vi "Semaphore Open.vi"(7 "permissions (0664)":T2={"owner"={"read"=TRUE, "write"=TRUE, "execute"=FALSE}, "group"={"read"=TRUE, "write"=TRUE, "execute"=FALSE}, "everyone"={"read"=TRUE, "write"=FALSE, "execute"=FALSE}}, 8 "error in (no error)":errorcluster, 9 "initial value (0)":u32, 10 "file mode (open)":T1, 11 "name":string) -> (0 "error out":errorcluster, 3 "Semaphore out":T3)   [LabVIEW 2016, in "Linux RT IPC.POSIX Threads.lvlib" / "Semaphore.lvclass"]
doc: "Calls sem_open() to open a reference to a named semaphore and returns a pointer.\n\nThis VI initializes the semaphore object and sets its default values.\n\nRefer to online POSIX documentation for more information."
uses:
  Semaphore.lvclass
  Controls/reference.ctl
  Shared Memory/Controls/file mode.ctl
  C/Controls/file creation flags.ctl
  POSIX Thread Object/Private VIs/libpthread path.vi
  C/SubVIs/permission group to mode_t.vi
  C/SubVIs/OR flags U32.vi
  POSIX Thread Object/Private VIs/get pthread error.vi
  <vilib>/NI/NI Linux RT Errno/VIs/Public/SubVIs/errno enum to number.vi
  <vilib>/NI/NI Linux RT Errno/VIs/Public/Get Errno Value for Calling Thread.vi
  POSIX Thread Object/POSIX Thread Object.lvclass
  C/Linux RT IPC.C.lvlib
  Shared Memory/Linux RT IPC.Shared Memory.lvlib
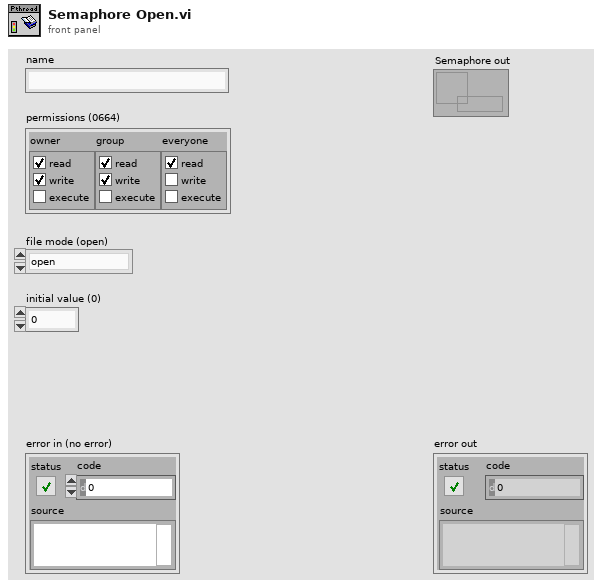
[diagram p1: front panel]
types:
  T1 = typedef "Linux RT IPC.Shared Memory.lvlib/file mode.ctl" = enum16{"open", "create/replace"}
  T2 = cluster{"owner":cluster{"read":bool, "write":bool, "execute":bool}, "group":cluster{"read":bool, "write":bool, "execute":bool}, "everyone":cluster{"read":bool, "write":bool, "execute":bool}}
  T3 = typedef "Linux RT IPC.POSIX Threads.lvlib/Semaphore.lvclass/reference.ctl" = refnum<data-value>
  T4 = typedef "Linux RT IPC.C.lvlib/file creation flags.ctl" = u32
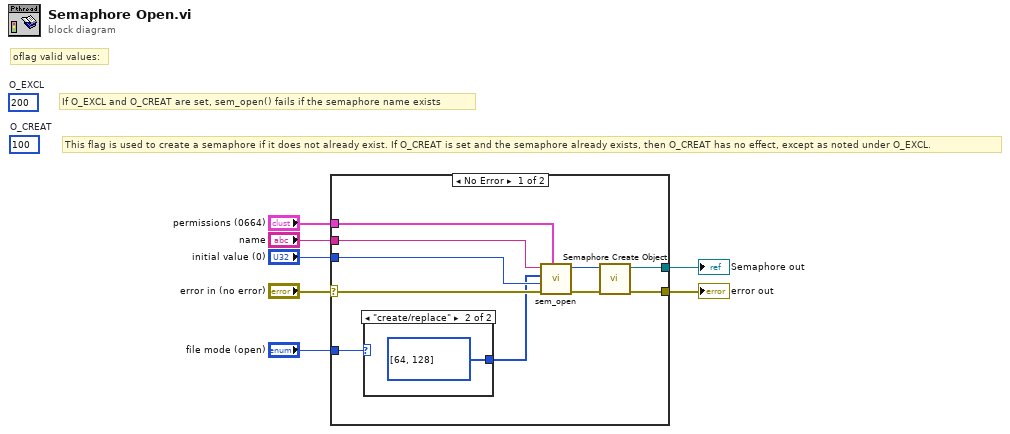
[diagram p0: block diagram]
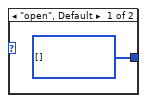
[diagram p2: hidden frame]
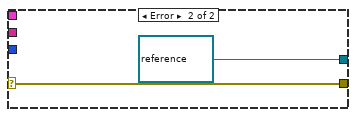
[diagram p3: hidden frame]
diagram:
  (unwired) u32 200  # O_EXCL
  (unwired) u32 100  # O_CREAT
  # "If O_EXCL and O_CREAT are set, sem_open() fails if the semaphore name exists"
  # "This flag is used to create a semaphore if it does not already exist. If O_CREAT is set and the semaphore already exists, then O_CREAT has no effect, except as noted under O_EXCL."
  # "oflag valid values:"
  n1 = case shown="No Error" "error in (no error)" {
    selector: "error in (no error)" -> [w15 w21]
    tunnel: [w11 w21] -> w6
    tunnel: "name" -> [w17 _]
    tunnel: "initial value (0)" -> [w16 _]
    tunnel: "permissions (0664)" -> [w14 _]
    tunnel: [w10 T3 refnum ("Semaphore out")] -> w2
    tunnel: "file mode (open)" -> [w9 _]
    frame No Error {
      n2 = case shown="\"create/replace\"" w9 {
        tunnel: [w18 w19] -> w8
        frame "open", Default {
          w18 = T4[] [] items=["O_RDONLY"=0, "O_WRONLY"=1, "O_RDWR"=2, "O_CREAT"=64, "O_EXCL"=128, "O_TRUNC"=512] ("file creation flags")
        }
        frame "create/replace" {
          w19 = T4[] [64, 128] items=["O_RDONLY"=0, "O_WRONLY"=1, "O_RDWR"=2, "O_CREAT"=64, "O_EXCL"=128, "O_TRUNC"=512] ("file creation flags")
        }
      }
      n3 = call "sem_open.vi"("permissions (0664)"=w14, "error in (no error)"=w15, "initial value (0)"=w16, "flags"=w8, "name"=w17) -> ("error out"=w13:errorcluster, "semaphore ptr out"=w12:u64)  [unwired: 5 in]
      n4 = call "Semaphore Create Object.vi"("error in (no error)"=w13, "semaphore pointer"=w12) -> ("error out"=w11:errorcluster, "Semaphore out"=w10:T3)  [unwired: 8 in]
    }
    frame Error {
    }
  }
  "error out" <- w6
  "Semaphore out" <- w2
